vi "DepositBins.vi"(1 "Port 2":T4 items=["Port 1", "Port 2", "Port 3", "Port 4"], 2 "Port 1":T4 items=["Port 1", "Port 2", "Port 3", "Port 4"], 3 "NXT/EV3 IN":T2, 4 "Movement Power":dbl, 5 "Turn Power":dbl, 6 "Motor IDs":cluster{"Motors":T1, "Motors 2":T1}={"Motors"=0, "Motors 2"=1} {"Motors 2" items=["Port A", "Port B", "Port C", "Port D"]; "Motors" items=["Port A", "Port B", "Port C", "Port D"]}, 7 "ColorH":T3=enum."Blue", 8 "ColorL":T3=enum."Blue", 10 "isHeavy":bool) -> (0 "NXT/EV3 OUT":T2, 9 "isDone":bool)   [LabVIEW 2016, in "13.03 Robot.lvrbt"]
uses:
  13.03 Robot.lvrbt
  <vilib>/NXT/Block Support/NXT_InputPort.ctl
  <vilib>/NXT/Subs/ColorSensorColors.ctl
  <vilib>/NXT/Subs/LVHSConnector.ctl
  <vilib>/NXT/LegoClasses/BrickReference/BrickReference.lvclass
  <vilib>/NXT/Block Support/NXT_OutputPort.ctl
  <vilib>/NXT/Dual Mode Library/Display/drawText.vi
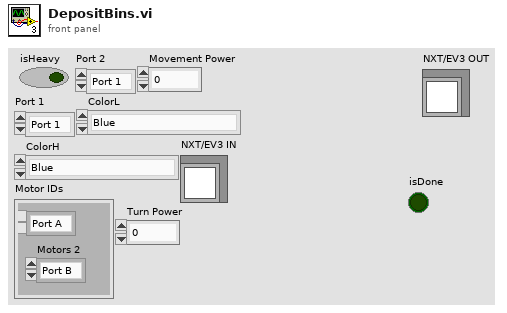
[diagram p1: front panel]
types:
  T1 = typedef "NXT_OutputPort.ctl" = u8
  T2 = typedef "LVHSConnector.ctl" = refnum<class "BrickReference.lvclass">
  T3 = typedef "ColorSensorColors.ctl" = enum16{"No Color", "Black", "Blue", "Green", "Yellow", "Red", "White", "Brown"}
  T4 = typedef "NXT_InputPort.ctl" = u32
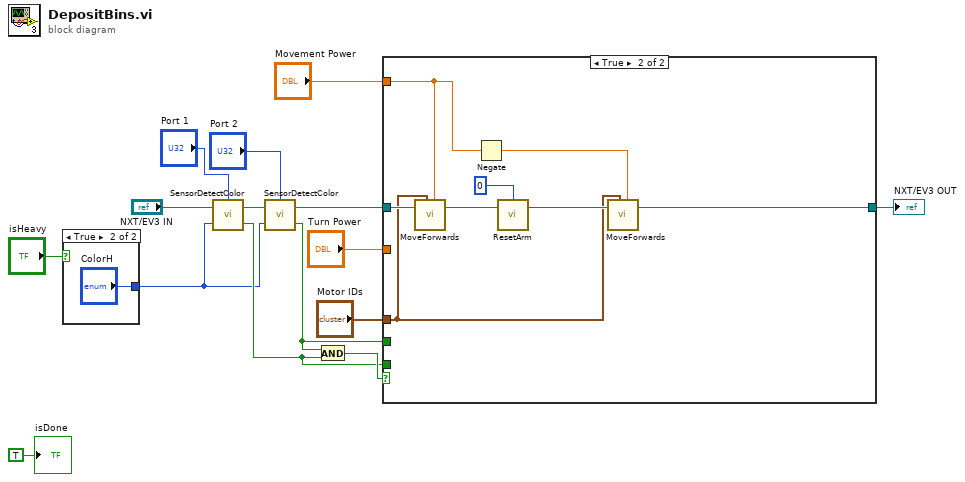
[diagram p0: block diagram]
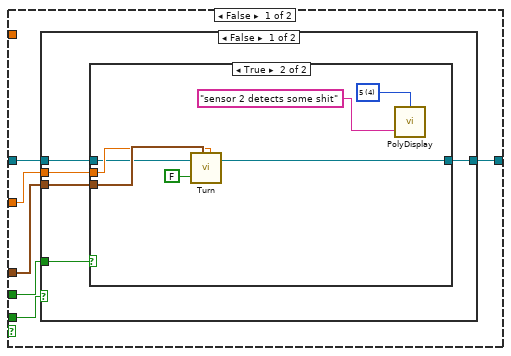
[diagram p2: hidden frame]
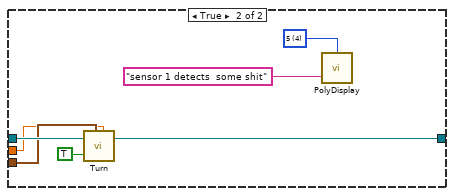
[diagram p4: hidden frame]
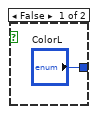
[diagram p5: hidden frame]
diagram:
  n1 = case shown="True" "isHeavy" {
    tunnel: ["ColorL" "ColorH"] -> w2
    frame False {
    }
    frame True {
    }
  }
  n2 = call "SensorDetectColor.vi"("Color"=w2, "NXT/EV3 IN"="NXT/EV3 IN", "Port"="Port 1") -> ("Out"=w6:bool, "NXT/EV3 OUT"=w11:T2)
  n3 = call "SensorDetectColor.vi"("Color"=w2, "NXT/EV3 IN"=w11, "Port"="Port 2") -> ("Out"=w4:bool, "NXT/EV3 OUT"=w8:T2)
  n4 = And(x=w4, y=w6) -> (x .and. y?=w10:bool)
  n5 = case shown="True" w10 {
    tunnel: "Motor IDs" -> [w21 w47]
    tunnel: w8 -> [w22 w51]
    tunnel: "Movement Power" -> [_ w46]
    tunnel: w6 -> [w23 _]
    tunnel: "Turn Power" -> [w20 _]
    tunnel: w4 -> [w19 _]
    tunnel: [w18 w44] -> w3
    frame False {
      n6 = case shown="False" w23 {
        tunnel: w22 -> [w25 w43]
        tunnel: w21 -> [w27 w42]
        tunnel: w20 -> [w26 w40]
        tunnel: w19 -> [w28 _]
        tunnel: [w24 w39] -> w18
        frame False {
          n7 = case shown="True" w28 {
            tunnel: w27 -> [_ w36]
            tunnel: w26 -> [_ w35]
            tunnel: w25 -> [w29 w34]
            tunnel: [w29 w32] -> w24
            frame False {
            }
            frame True {
              w30 = i16 4 items=["1", "2", "3", "4", "5", "6", "7", "8", "9", "10", "11", "12"] ("Line")
              n8 = call "Turn.vi"("T - 1st, F - 2nd"=FALSE, "NXT/EV3 IN"=w34, "Motor IDs"=w36, "Power"=w35) -> ("NXT/EV3 OUT"=w32:T2)
              n9 = call-poly <vilib>:"PolyDisplay.vi"("Text"="sensor 2 detects some shit", "Line"=w30) -> ()  [unwired: 2 in, 1 out]
            }
          }
        }
        frame True {
          w38 = i16 4 items=["1", "2", "3", "4", "5", "6", "7", "8", "9", "10", "11", "12"] ("Line")
          n10 = call "Turn.vi"("T - 1st, F - 2nd"=TRUE, "NXT/EV3 IN"=w43, "Motor IDs"=w42, "Power"=w40) -> ("NXT/EV3 OUT"=w39:T2)
          n11 = call-poly <vilib>:"PolyDisplay.vi"("Text"="sensor 1 detects  some shit", "Line"=w38) -> ()  [unwired: 2 in, 1 out]
        }
      }
    }
    frame True {
      n12 = call "MoveForwards.vi"("NXT/EV3 IN"=w51, "Motor IDs"=w47, "Power"=w46) -> ("NXT/EV3 OUT"=w50:T2)  [unwired: 1 in]
      n13 = Negate(x=w46) -> (-x=w45:dbl)
      n14 = call "ResetArm.vi"("NXT/EV3 IN"=w50, "ResetTo"=0) -> ("NXT/EV3 OUT"=w48:T2)  [unwired: 1 in]
      n15 = call "MoveForwards.vi"("NXT/EV3 IN"=w48, "Motor IDs"=w47, "Power"=w45) -> ("NXT/EV3 OUT"=w44:T2)  [unwired: 1 in]
    }
  }
  "NXT/EV3 OUT" <- w3
  "isDone" <- TRUE ("isDone")
